vi "Create.vi"(5 "Test Executor in":refnum<class "Test Executor.lvclass">, 8 "error in (no error)":errorcluster, 10 "Result Queue (none)":refnum<queue>, 11 "Application":refnum<vi>) -> (0 "error out":errorcluster, 3 "Test Executor":refnum<class "Test Executor.lvclass">)   [LabVIEW 2017, in "Test Executor.lvclass"]
uses:
  Test Executor.lvclass
  Test Result/Test Result.lvclass
  Test Executor.lvclass/Test Executor.ctl
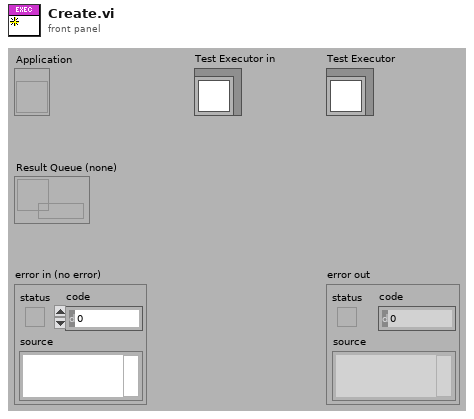
[diagram p1: front panel]
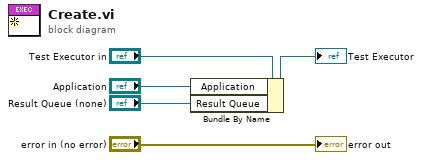
[diagram p0: block diagram]
diagram:
  n1 = Bundle By Name(cluster="Test Executor in", "Application"="Application", "Result Queue"="Result Queue (none)") -> (→"Test Executor":refnum<class "Test Executor.lvclass">)
  "error out" <- "error in (no error)"
